vi "LookupMethod.vi"(9 "Method Paths":path[](array[path]), 10 "Fully Qualified Method Names":string[](array[string]), 11 "Command":string) -> (2 "Found?":bool, 3 "Method Path":path)   [LabVIEW 2019, in "MicronServer.lvlib" / "Mapper.lvclass"]
uses:
  Mapper.lvclass
  Typedefs/VIMatchType.ctl
  <vilib>/SLL Toolkit/SLL String/_SubVIs/Search 1D String Array First Match.vi
  <vilib>/SLL Toolkit/SLL String/SLL String.lvlib
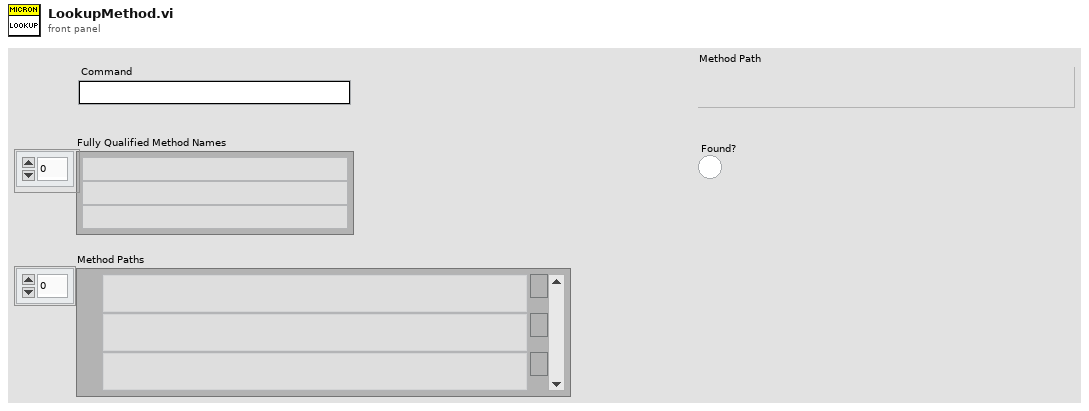
[diagram p1: front panel]
types:
  T1 = typedef "MicronServer.lvlib/Mapper.lvclass/VIMatchType.ctl" = enum16{"Full Match", "VI File Name with Ext", "VI File Name without Ext", "VI File Name Partial Match", "Partial Match"}
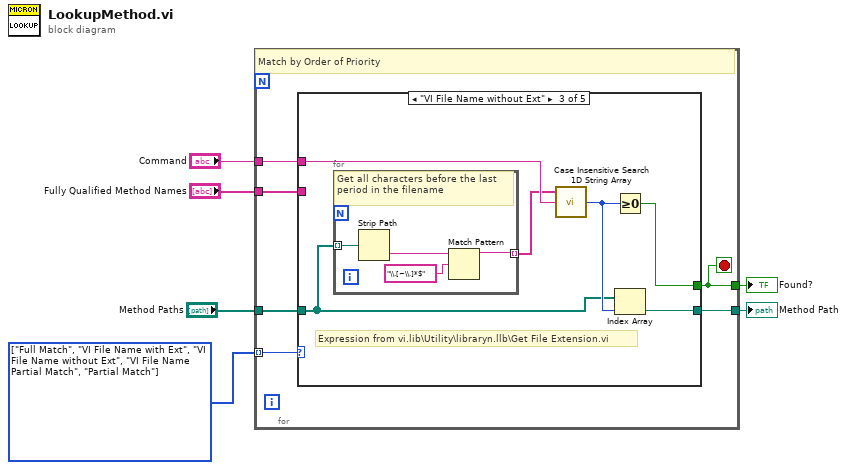
[diagram p0: block diagram]
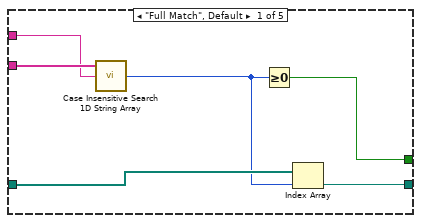
[diagram p2: hidden frame]
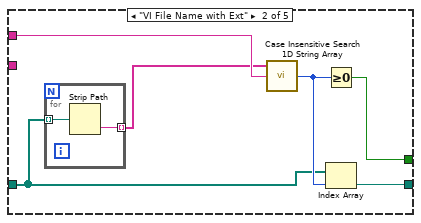
[diagram p3: hidden frame]
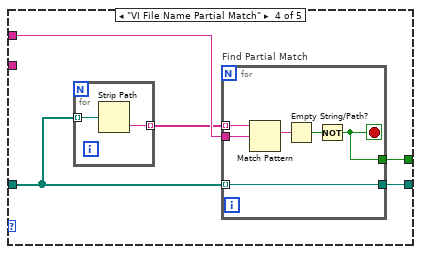
[diagram p4: hidden frame]
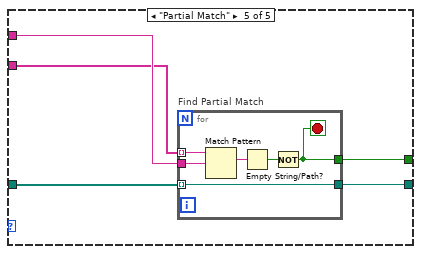
[diagram p5: hidden frame]
diagram:
  w1 = T1[] [enum."Full Match", enum."VI File Name with Ext", enum."VI File Name without Ext", enum."VI File Name Partial Match", enum."Partial Match"] items=["Full Match", "VI File Name with Ext", "VI File Name without Ext", "VI File Name Partial Match", "Partial Match"]
  n1 = for {
    tunnel: [w8] -> w6
    tunnel: [w12] -> w5
    tunnel: "Command" -> [w11]
    tunnel: "Method Paths" -> [w10]
    tunnel: "Fully Qualified Method Names" -> [w9]
    tunnel: w1 -> [w7] mode=indexing
    stop <- w8 stop-if-true
    # "Match by Order of Priority"
    n2 = case shown="\"VI File Name without Ext\"" w7 {
      tunnel: [w16 w23 w31 w41 w54] -> w8
      tunnel: [w13 w21 w29 w40 w53] -> w12
      tunnel: w11 -> [w17 w24 w32 w39 w52]
      tunnel: w10 -> [w15 w20 w28 w38 w51]
      tunnel: w9 -> [w18 _ _ _ w50]
      frame "Full Match", Default {
        n3 = call-poly <vilib>:"Case Insensitive Search 1D String Array.vi"("Element"=w17, "1D String Array"=w18) -> ("Index"=w14:i32)  [unwired: 1 in]
        n4 = Greater Or Equal To 0?(x=w14) -> (x >= 0?=w16:bool)
        n5 = Index Array(array=w15, index=w14) -> (element=w13:path)
      }
      frame "VI File Name with Ext" {
        n6 = for {
          tunnel: w20 -> [w26] mode=indexing
          tunnel: [w25] -> w19 mode=indexing
          n7 = Strip Path(path=w26) -> (name=w25:string)  [unwired: 1 out]
        }
        n8 = call-poly <vilib>:"Case Insensitive Search 1D String Array.vi"("Element"=w24, "1D String Array"=w19) -> ("Index"=w22:i32)  [unwired: 1 in]
        n9 = Greater Or Equal To 0?(x=w22) -> (x >= 0?=w23:bool)
        n10 = Index Array(array=w20, index=w22) -> (element=w21:path)
      }
      frame "VI File Name without Ext" {
        # "Expression from vi.lib\\Utility\\libraryn.llb\\Get File Extension.vi"
        n11 = for {
          tunnel: w28 -> [w36] mode=indexing
          tunnel: [w33] -> w27 mode=indexing
          # "Get all characters before the last period in the filename"
          n12 = Strip Path(path=w36) -> (name=w35:string)  [unwired: 1 out]
          n13 = Match Pattern(string=w35, regular expression="\\.[~\\.]*$") -> (before substring=w33:string)  [unwired: 4 out]
        }
        n14 = call-poly <vilib>:"Case Insensitive Search 1D String Array.vi"("Element"=w32, "1D String Array"=w27) -> ("Index"=w30:i32)  [unwired: 1 in]
        n15 = Greater Or Equal To 0?(x=w30) -> (x >= 0?=w31:bool)
        n16 = Index Array(array=w28, index=w30) -> (element=w29:path)
      }
      frame "VI File Name Partial Match" {
        n17 = for {
          tunnel: w38 -> [w43] mode=indexing
          tunnel: [w42] -> w37 mode=indexing
          n18 = Strip Path(path=w43) -> (name=w42:string)  [unwired: 1 out]
        }
        n19 = for "Find Partial Match" {
          tunnel: w37 -> [w49] mode=indexing
          tunnel: w38 -> [w45] mode=indexing
          tunnel: w39 -> [w48]
          tunnel: [w45] -> w40
          tunnel: [w44] -> w41
          stop <- w44 stop-if-true
          n20 = Match Pattern(string=w49, regular expression=w48) -> (match substring=w47:string)  [unwired: 1 in, 3 out]
          n21 = Empty String/Path?(string/path=w47) -> (empty?=w46:bool)
          n22 = Not(x=w46) -> (.not. x?=w44:bool)
        }
      }
      frame "Partial Match" {
        n23 = for "Find Partial Match" {
          tunnel: w50 -> [w60] mode=indexing
          tunnel: w51 -> [w56] mode=indexing
          tunnel: w52 -> [w59]
          tunnel: [w56] -> w53
          tunnel: [w55] -> w54
          stop <- w55 stop-if-true
          n24 = Match Pattern(string=w60, regular expression=w59) -> (match substring=w58:string)  [unwired: 1 in, 3 out]
          n25 = Empty String/Path?(string/path=w58) -> (empty?=w57:bool)
          n26 = Not(x=w57) -> (.not. x?=w55:bool)
        }
      }
    }
  }
  "Found?" <- w6
  "Method Path" <- w5
